vi "Panel.vi"(11 "Panel In":refnum<class "DeviceDetailPanel.lvclass">) -> ()   [LabVIEW 2020, in "PicoG-App.lvlib" / "DeviceDetailPanel.lvclass"]
uses:
  DeviceDetailPanel.lvclass
  C:/Program Files (x86)/National Instruments/LabVIEW 2020/vi.lib/IlluminatedG/IG OOPanel/OOPanel/Panel/Panel.lvclass
  <vilib>/IlluminatedG/IG OOPanel/OOPanel/Panel/Basic UI State.ctl
  Terminal State.ctl
  DeviceDetailPanel.lvclass/DeviceDetailPanel.ctl
  ViaApp/ViaApp.lvclass
  Device/Device.lvclass
  Builds/picoG/ppl/PicoG-Core.lvlibp/PicoG-Processor/PicoG-Core/Platform/Platform.lvclass
  <vilib>/IlluminatedG/IG OOPanel/OOPanel/Panel/Panel.lvclass
  <vilib>/IlluminatedG/IG OOPanel/OOPanel/OOPanel.lvlib
  C:/dev/picoG/PicoG/PicoG-App/DeviceDetailPanel/DeviceDetailPanel.lvclass
  Builds/picoG/ppl/PicoG-Core.lvlibp/PicoG-Processor/PicoG-Core/Resource/Resource.lvclass
panel:
  in  "Remove":bool
  out "Alias":string
  in  "Set Alias":bool
  out "Resource":string
  out "Picture":picture
  out "Version":string
  out "Board":string
  out "Platform":string
  out "ID":string
  out "Device Status":string="Unknown"
  out "Terminal Status":string
  in  "Close":bool
  in  "Open":bool
  out "Terminal Underlay":string
  # "Platform"
  # "Board"
  # "Serial"
  # "Version"
  # "Resource"
  # "Status"
  # "Terminal"
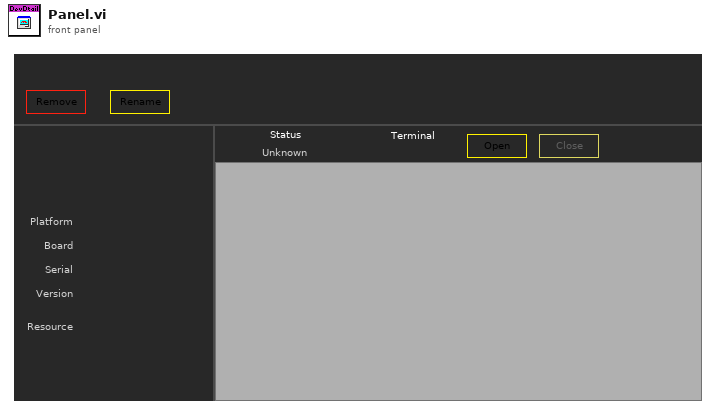
[diagram p1: front panel]
types:
  T1 = typedef "OOPanel.lvlib/Panel.lvclass/Basic UI State.ctl" = enum16{"Init", "Run", "Close"}
  T2 = typedef "PicoG-App.lvlib/DeviceDetailPanel.lvclass/Terminal State.ctl" = enum16{"Disconnected", "Connecting", "Connected", "Error"}
  T3 = enum8{"Enabled", "Disabled", "Disabled and Grayed Out"}
  T4 = typedef "PicoG-App.lvlib/DeviceDetailPanel.lvclass/Inbound Events.ctl" = cluster{"Device Updated":refnum<user-event>, "Deploy":refnum<user-event>}
  T5 = typedef "OOPanel.lvlib/Panel.lvclass/Panel Events.ctl" = cluster{"Visbility":refnum<user-event>, "Close":refnum<user-event>}
  T6 = typedef "PicoG-App.lvlib/DeviceDetailPanel.lvclass/Ref Data.ctl" = cluster{"Device":refnum<class "Device.lvclass">}
  T7 = typedef "OOPanel.lvlib/Panel.lvclass/Visibility State.ctl" = enum16{"Idle", "Closed", "Hidden", "Visible", "Subpanel"}
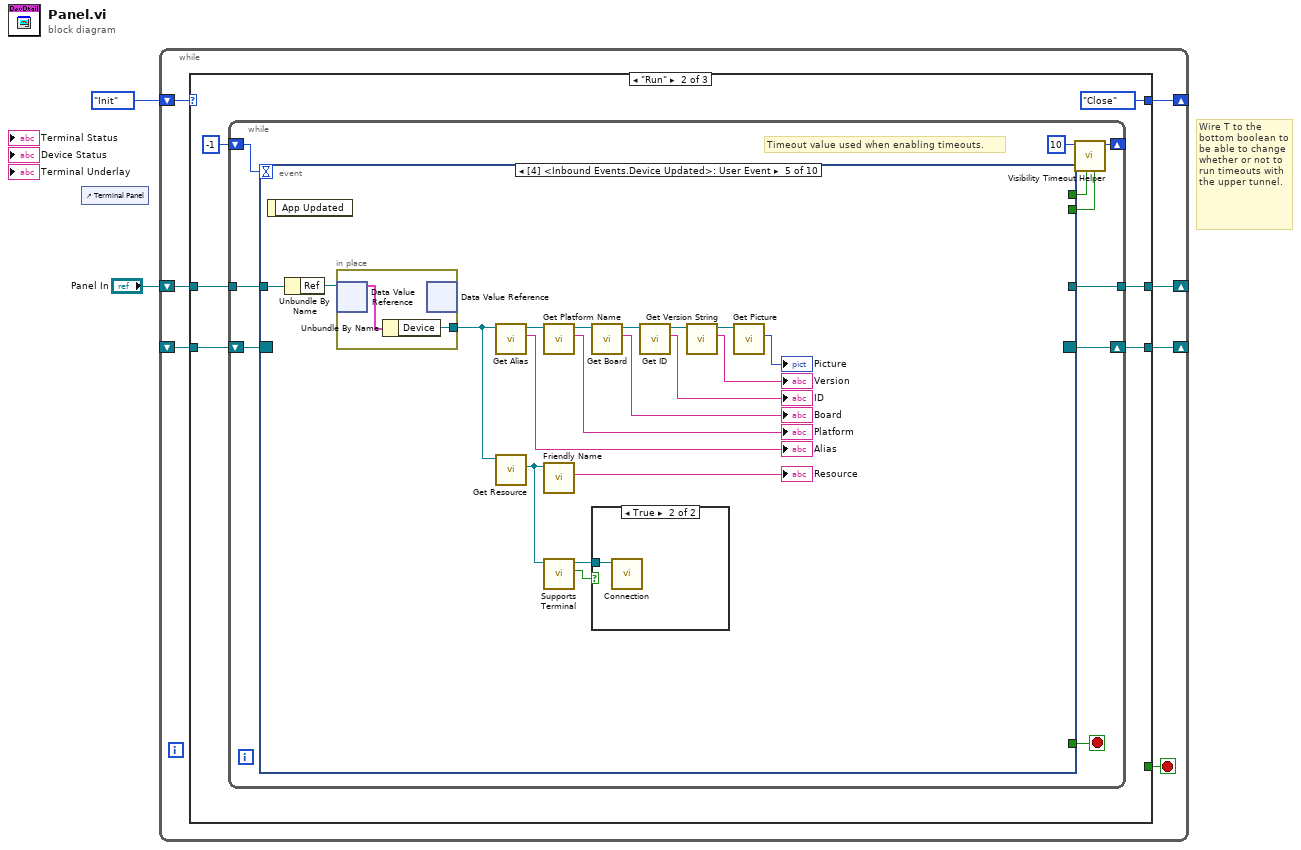
[diagram p0: block diagram]
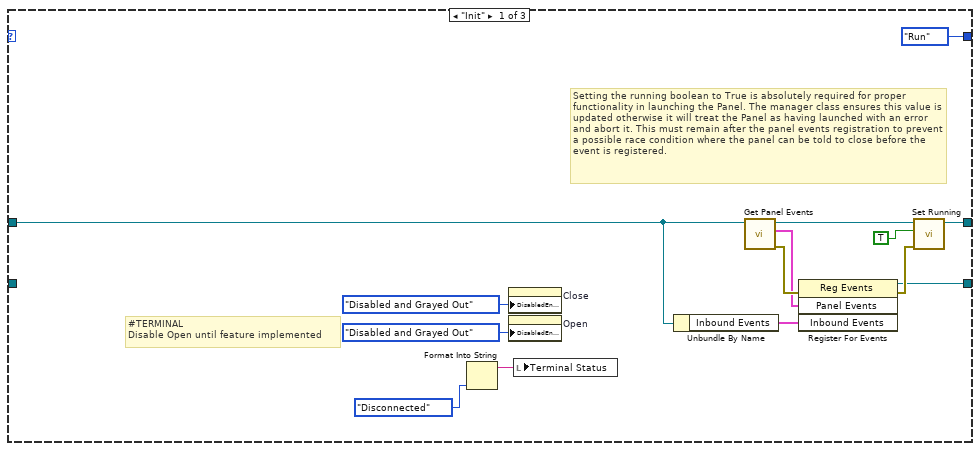
[diagram p2: hidden frame]
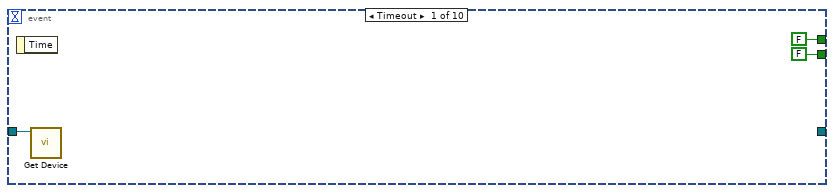
[diagram p3: hidden frame]
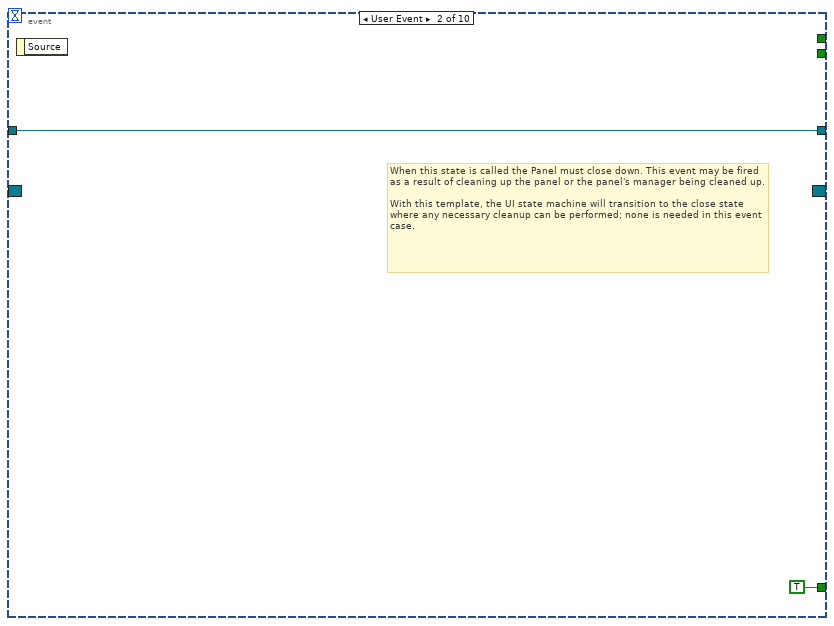
[diagram p4: hidden frame]
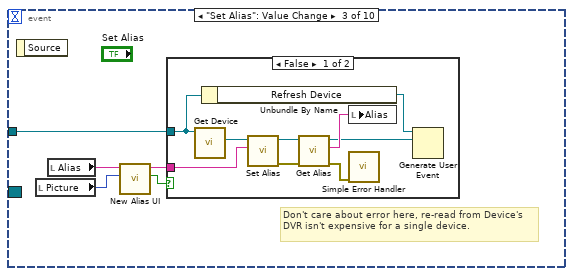
[diagram p5: hidden frame]
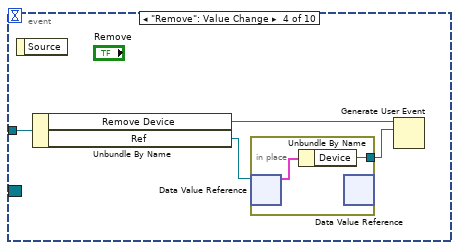
[diagram p7: hidden frame]
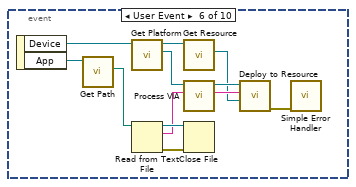
[diagram p9: hidden frame]
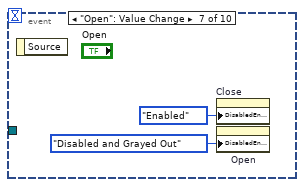
[diagram p10: hidden frame]
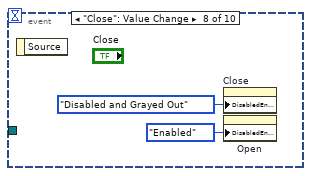
[diagram p11: hidden frame]
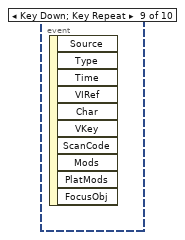
[diagram p12: hidden frame]
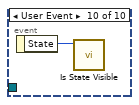
[diagram p13: hidden frame]
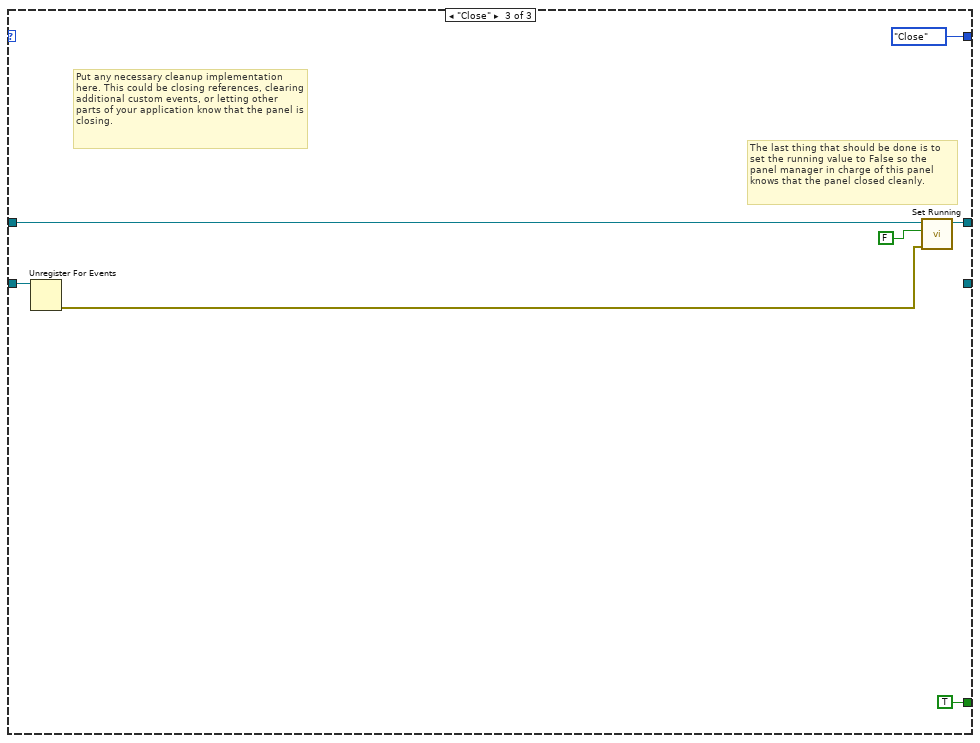
[diagram p14: hidden frame]
diagram:
  # "Wire T to the bottom boolean to be able to change whether or not to run timeouts with the upper tunnel."
  n1 = control-ref of="Terminal Panel"() -> ()  [unwired: 1 out]
  n2 = while {
    shift-right: [w8] -> _
    shift-left: _ -> [w9]
    shift-right: [w6] -> _
    shift-left: Basic_UI_State."Init" ("Basic UI State") -> [w7]
    shift-right: [w4] -> _
    shift-left: "Panel In" -> [w3]
    stop <- w5 stop-if-true
    n3 = case shown="\"Run\"" w7 {
      tunnel: w9 -> [_ w29 w105]
      tunnel: [w17 w27 _] -> w8
      tunnel: [Basic_UI_State."Run" ("Basic UI State") Basic_UI_State."Close" ("Basic UI State") Basic_UI_State."Close" ("Basic UI State")] -> w6
      tunnel: [_ _ TRUE] -> w5
      tunnel: [w16 w24 w103] -> w4
      tunnel: w3 -> [w11 w25 w104]
      frame "Init" {
        # "#TERMINAL\nDisable Open until feature implemented"
        # "Setting the running boolean to True is absolutely required for proper functionality in launching the Panel. The manager class ensures this value is updated otherwise it will treat the Panel as having launched with an error and abort it. This must remain after the panel events registration to prevent a possible race condition where the panel can be told to close before the event is registered."
        n4 = Format Into String(Terminal_State."Disconnected" ("Terminal State")) -> (resulting string=w13:string)  [unwired: 3 in, 1 out]
        n5 = property on="Close" class="Bool"("DisabledEnum"=T3."Disabled and Grayed Out" ("Disabled")) -> ()  [unwired: 2 in, 2 out]
        n6 = property on="Open" class="Bool"("DisabledEnum"=T3."Disabled and Grayed Out" ("Disabled")) -> ()  [unwired: 2 in, 2 out]
        n7 = local write "Terminal Status"(w13) -> ()
        n8 = Unbundle By Name(w11) -> ("Inbound Events"=w10:T4)
        n9 = call <vilib>:"Get Panel Events.vi"("Panel in"=w11) -> ("error out"=w23:errorcluster, "Panel Events"=w19:T5, "Panel out"=w20:refnum<class "DeviceDetailPanel.lvclass">)  [unwired: 8 in]
        n10 = register-events(error in=w23, w19, w10) -> (reference out=w17:refnum<event-registration>, error out=w21:errorcluster)  [unwired: 1 in]
        n11 = call <vilib>:"Set Running.vi"("error in (no error)"=w21, "Running"=TRUE, "Panel in"=w20) -> ("Panel out"=w16:refnum<class "DeviceDetailPanel.lvclass">)  [unwired: 7 in, 1 out]
      }
      frame "Run" {
        n12 = while {
          shift-right: [w35] -> w27
          shift-left: w29 -> [w36]
          shift-right: [w38] -> _
          shift-left: -1 ("Timeout") -> [w37]
          tunnel: w25 -> [w31]
          tunnel: [w30] -> w24
          stop <- w32 stop-if-true
          # "Timeout value used when enabling timeouts."
          n13 = event shown="[4] <Inbound Events.Device Updated>: User Event" {
            selector: w36 -> [_ _ _ _ _ _ _ _ _ _]
            dyn-events: [_ _ _ _ _ _ _ _ _ _] -> w35
            timeout: w37 -> [_ _ _ _ _ _ _ _ _ _]
            tunnel: [FALSE _ _ _ _ _ _ _ _ _] -> w34
            tunnel: [FALSE _ _ _ _ _ _ _ _ _] -> w33
            tunnel: [_ TRUE _ _ _ _ _ _ _ _] -> w32
            tunnel: w31 -> [w40 w43 w46 w61 w81 _ _ _ _ _]
            tunnel: [_ w43 _ _ _ _ _ _ _ _] -> w30
            event Timeout {
              n14 = event-data() -> ()  [unwired: 1 in, 1 out]
              n15 = call "Get Device.vi"("DeviceDetailPanel in"=w40) -> ()  [unwired: 8 in, 3 out]
            }
            event User Event {
              # "When this state is called the Panel must close down. This event may be fired as a result of cleaning up the panel or the panel's manager being cleaned up.\n\nWith this template, the UI state machine will transition to the close state where any necessary cleanup can be performed; none is needed in this event case."
              n16 = event-data() -> ()  [unwired: 1 in, 1 out]
            }
            event "Set Alias": Value Change {
              # "Don't care about error here, re-read from Device's DVR isn't expensive for a single device."
              n17 = event-data() -> ()  [unwired: 1 in, 1 out]
              n18 = local read "Picture"() -> (w45:picture)
              n19 = local read "Alias"() -> (w48:string)
              n20 = call "New Alias UI.vi"("Picture"=w45, "Current Alias"=w48) -> ("Cancelled"=w49:bool, "Alias"=w47:string)  [unwired: 8 in]
              n21 = case shown="False" w49 {
                tunnel: w47 -> [w57 _]
                tunnel: w46 -> [w52 _]
                frame False {
                  n22 = call "Get Device.vi"("DeviceDetailPanel in"=w52) -> ("Device"=w58:refnum<class "Device.lvclass">)  [unwired: 8 in, 2 out]
                  n23 = Unbundle By Name(w52) -> ("Refresh Device"=w51:refnum<user-event>)
                  n24 = call "Set Alias.vi"("Alias"=w57, "Device in"=w58) -> ("error out"=w55:errorcluster, "Device out"=w56:refnum<class "Device.lvclass">)  [unwired: 8 in]
                  n25 = call "Get Alias.vi"("error in (no error)"=w55, "Device in"=w56) -> ("error out"=w53:errorcluster, "Alias"=w54:string, "Device out"=w50:refnum<class "Device.lvclass">)  [unwired: 7 in]
                  n26 = local write "Alias"(w54) -> ()
                  n27 = call <vilib>:"Simple Error Handler.vi"("error in (no error)"=w53) -> ()  [unwired: 4 in, 5 out]
                  n28 = Generate User Event(user event=w51, event data cluster=w50) -> ()  [unwired: 2 in, 2 out]
                }
                frame True {
                }
              }
            }
            event "Remove": Value Change {
              n29 = event-data() -> ()  [unwired: 1 in, 1 out]
              n30 = Unbundle By Name(w61) -> ("Remove Device"=w60:refnum<user-event>, "Ref"=w62:refnum<data-value>)
              n31 = in-place {
                in-place-border: [w63] -> w59
                n32 = in-place-dvr #1(w62) -> (w64:T6)  [unwired: 1 out]
                n33 = Unbundle By Name(w64) -> ("Device"=w63:refnum<class "Device.lvclass">)
                n34 = in-place-dvr #1() -> ()  [unwired: 1 in, 2 out]
              }
              n35 = Generate User Event(user event=w60, event data cluster=w59) -> ()  [unwired: 2 in, 2 out]
            }
            event User Event {
              n36 = event-data() -> ()  [unwired: 1 in, 1 out]
              n37 = Unbundle By Name(w81) -> ("Ref"=w82:refnum<data-value>)
              n38 = in-place {
                in-place-border: [w84] -> w69
                n39 = in-place-dvr #2(w82) -> (w85:T6)  [unwired: 1 out]
                n40 = Unbundle By Name(w85) -> ("Device"=w84:refnum<class "Device.lvclass">)
                n41 = in-place-dvr #2() -> ()  [unwired: 1 in, 2 out]
              }
              n42 = call "Get Alias.vi"("Device in"=w69) -> ("Alias"=→"Alias":string, "Device out"=w79:refnum<class "Device.lvclass">)  [unwired: 8 in, 1 out]
              n43 = call "Get Resource.vi"("Device in"=w69) -> ("Resource"=w67:refnum<class "Resource.lvclass">)  [unwired: 8 in, 2 out]
              n44 = call "Get Platform Name.vi"("Device in"=w79) -> ("Platform"=→"Platform":string, "Device out"=w77:refnum<class "Device.lvclass">)  [unwired: 8 in, 1 out]
              n45 = call-dynamic "Friendly Name.vi"("DeployResource in"=w67) -> ("Friendly Name"=→"Resource":string)  [unwired: 8 in, 2 out]
              n46 = call-dynamic "Supports Terminal.vi"("Resource in"=w67) -> ("Supports Terminal"=w65:bool, "Resource out"=w66:refnum<class "Resource.lvclass">)  [unwired: 8 in, 1 out]
              n47 = call "Get Board.vi"("Device in"=w77) -> ("Board"=→"Board":string, "Device out"=w75:refnum<class "Device.lvclass">)  [unwired: 8 in, 1 out]
              n48 = case shown="True" w65 {
                tunnel: w66 -> [_ w83]
                frame False {
                }
                frame True {
                  n49 = call-dynamic "Connection.vi"("Resource in"=w83) -> ()  [unwired: 8 in, 3 out]
                }
              }
              n50 = call "Get ID.vi"("Device in"=w75) -> ("Id"=→"ID":string, "Device out"=w73:refnum<class "Device.lvclass">)  [unwired: 8 in, 1 out]
              n51 = call "Get Version String.vi"("Device in"=w73) -> ("Version"=→"Version":string, "Device out"=w71:refnum<class "Device.lvclass">)  [unwired: 8 in, 1 out]
              n52 = call "Get Picture.vi"("Device in"=w71) -> ("Picture"=→"Picture":picture)  [unwired: 8 in, 2 out]
            }
            event User Event {
              n53 = event-data() -> ("Device"=w97:refnum<class "Device.lvclass">, "App"=w88:refnum<class "ViaApp.lvclass">)  [unwired: 1 in]
              n54 = call "Get Path.vi"("ViaApp in"=w88) -> ("Path"=w86:path)  [unwired: 8 in, 2 out]
              n55 = call "Get Platform.vi"("Device in"=w97) -> ("Platform"=w95:refnum<class "Platform.lvclass">, "Device out"=w96:refnum<class "Device.lvclass">)  [unwired: 8 in, 1 out]
              n56 = Read from Text File(file (use dialog)=w86) -> (refnum out=w90:refnum<file>, text=w87:string, error out=w89:errorcluster)  [unwired: 3 in, 1 out]
              n57 = call "Get Resource.vi"("Device in"=w96) -> ("Resource"=w92:refnum<class "Resource.lvclass">)  [unwired: 8 in, 2 out]
              n58 = call-dynamic "Process VIA.vi"("Raw VIA"=w87, "DeployTarget in"=w95) -> ("VIA"=w93:string, "DeployTarget out"=w94:refnum<class "Platform.lvclass">)  [unwired: 7 in, 1 out]
              n59 = Close File(refnum=w90, error in=w89) -> ()  [unwired: 2 out]
              n60 = call-dynamic "Deploy to Resource.vi"("Resource"=w92, "VIA"=w93, "DeployTarget in"=w94) -> ("error out"=w91:errorcluster)  [unwired: 6 in, 2 out]
              n61 = call <vilib>:"Simple Error Handler.vi"("error in (no error)"=w91) -> ()  [unwired: 4 in, 5 out]
            }
            event "Open": Value Change {
              n62 = event-data() -> ()  [unwired: 1 in, 1 out]
              n63 = property on="Close" class="Bool"("DisabledEnum"=T3."Enabled" ("Disabled")) -> ()  [unwired: 2 in, 2 out]
              n64 = property on="Open" class="Bool"("DisabledEnum"=T3."Disabled and Grayed Out" ("Disabled")) -> ()  [unwired: 2 in, 2 out]
            }
            event "Close": Value Change {
              n65 = event-data() -> ()  [unwired: 1 in, 1 out]
              n66 = property on="Close" class="Bool"("DisabledEnum"=T3."Disabled and Grayed Out" ("Disabled")) -> ()  [unwired: 2 in, 2 out]
              n67 = property on="Open" class="Bool"("DisabledEnum"=T3."Enabled" ("Disabled")) -> ()  [unwired: 2 in, 2 out]
            }
            event Key Down; Key Repeat {
              n68 = event-data() -> ()  [unwired: 1 in, 10 out]
            }
            event User Event {
              n69 = event-data() -> ("State"=w102:T7)  [unwired: 1 in]
              n70 = call <vilib>:"Is State Visible.vi"("Visibility"=w102) -> ()  [unwired: 10 in, 1 out]
            }
          }
          n71 = call <vilib>:"Visibility Timeout Helper.vi"("Update?"=w33, "Use Timeout?"=w34, "Visible Timeout mS"=10) -> ("Timeout"=w38:i32)  [unwired: 8 in]
        }
      }
      frame "Close" {
        # "Put any necessary cleanup implementation here. This could be closing references, clearing additional custom events, or letting other parts of your application know that the panel is closing."
        # "The last thing that should be done is to set the running value to False so the panel manager in charge of this panel knows that the panel closed cleanly."
        n72 = Unregister For Events(event registration refnum=w105) -> (error out=w107:errorcluster)  [unwired: 1 in]
        n73 = call <vilib>:"Set Running.vi"("error in (no error)"=w107, "Running"=FALSE, "Panel in"=w104) -> ("Panel out"=w103:refnum<class "DeviceDetailPanel.lvclass">)  [unwired: 7 in, 1 out]
      }
    }
  }
